vi "Find Chassis.vi"(6 "Map":map{string, T1}(c390), 11 "Hardware Type":T2) -> (2 "Chassis Info":T1, 3 "Has Chassis":bool)   [LabVIEW 2020, in "Volatus.lvlib" / "Hardware Info Module.lvclass"]
uses:
  Hardware Info Module.lvclass
  HW Info.ctl
  Hardware Type.ctl
  Hardware Info Module.lvclass/Hardware Info Module.ctl
  Volatus.lvlib
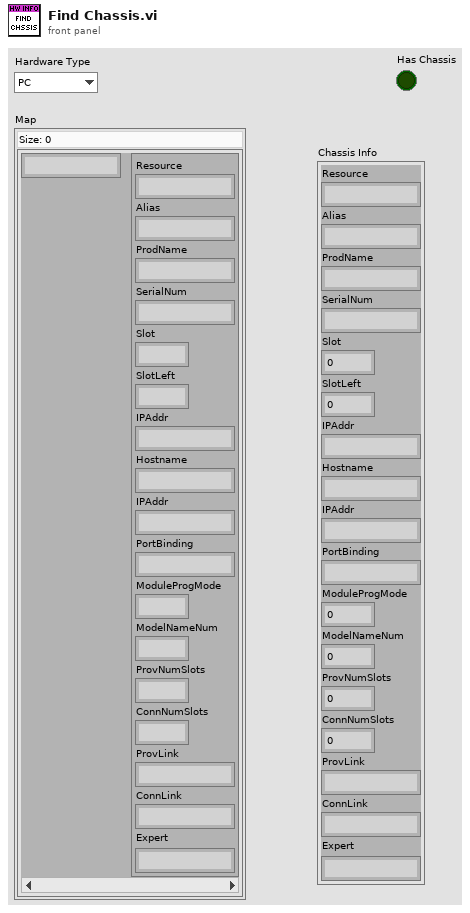
[diagram p1: front panel]
types:
  T1 = typedef "Volatus.lvlib/Hardware Info Module.lvclass/HW Info.ctl" = cluster{"Resource":string, "Alias":string, "ProdName":string, "SerialNum":string, "Slot":i32, "SlotLeft":u32, "IPAddr":string, "Hostname":string, "IPAddr":string, "PortBinding":string, "ModuleProgMode":u32, "ModelNameNum":u32, "ProvNumSlots":i32, "ConnNumSlots":i32, "ProvLink":string, "ConnLink":string, "Expert":string}
  T2 = typedef "Volatus.lvlib/Hardware Type.ctl" = enum16{"PC", "cRIO", "PXI"}
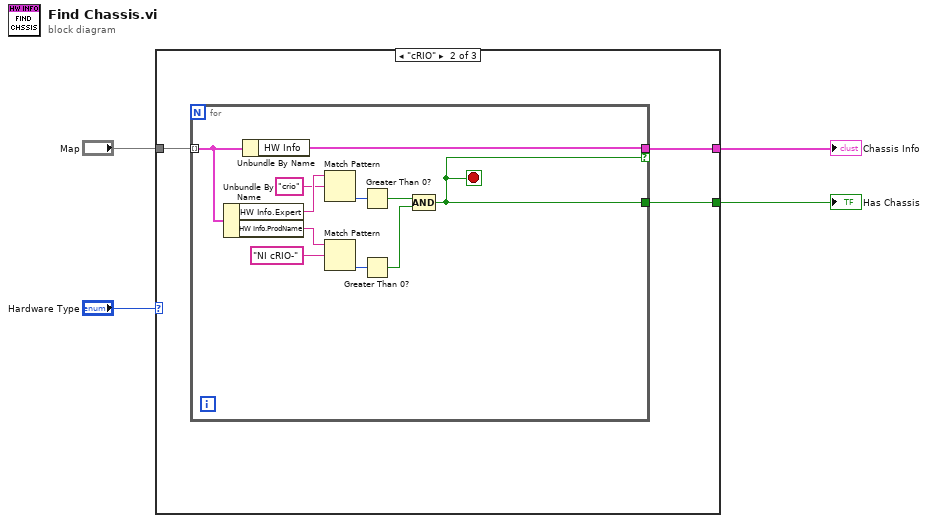
[diagram p0: block diagram]
diagram:
  n1 = case shown="\"cRIO\"" "Hardware Type" {
    tunnel: [_ w5 _] -> w3
    tunnel: "Map" -> [_ w7 _]
    tunnel: [_ w6 _] -> w1
    frame "PC" {
      # "#TODO\nCheck for MXI expansion"
    }
    frame "cRIO" {
      n2 = for {
        tunnel: w7 -> [w10] mode=indexing
        tunnel: [w9] -> w6 if=w8
        tunnel: [w8] -> w5
        stop <- w8 stop-if-true
        n3 = Unbundle By Name(w10) -> ("HW Info.Expert"=w18:string, "HW Info.ProdName"=w16:string)
        n4 = Unbundle By Name(w10) -> ("HW Info"=w9:T1)
        n5 = Match Pattern(string=w18, regular expression="crio") -> (offset past match=w13:i32)  [unwired: 1 in, 3 out]
        n6 = Match Pattern(string=w16, regular expression="NI cRIO-") -> (offset past match=w14:i32)  [unwired: 1 in, 3 out]
        n7 = Greater Than 0?(x=w13) -> (x > 0?=w12:bool)
        n8 = Greater Than 0?(x=w14) -> (x > 0?=w11:bool)
        n9 = Compound Arithmetic op=AND(w12, w11) -> (w8:bool)
      }
    }
    frame "PXI" {
    }
  }
  "Has Chassis" <- w3
  "Chassis Info" <- w1
